vi "Conpane Probe C.vi"(1 "x":dbl=1.0, 2 "factor":dbl=2.0) -> (0 "y":dbl)   [LabVIEW 2026]
doc: "Round-13 connector-pane probe: y = x * factor. Identical in all four variants; only conIdx differs, so any difference in the connector pane is caused by conIdx and nothing else."
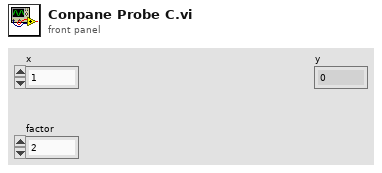
[diagram p1: front panel]
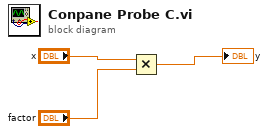
[diagram p0: block diagram]
diagram:
  n1 = Multiply(x="x", y="factor") -> (x*y=→"y":dbl)
